vi "Network Streams Chat Window Launcher Client.vi"() -> ()   [LabVIEW 2020]
uses:
  Chat Window/Chat Window.lvclass
  C:/Program Files/National Instruments/LabVIEW 2026/vi.lib/ActorFramework/Actor/Actor.lvclass
  Protocols/Network Stream Strategy/Network Stream/Network Stream.lvclass/Network Stream.ctl
  Protocols/Network Stream Strategy/Network Stream Initiator/Network Stream Initiator.lvclass/Network Stream Initiator.ctl
  Chat Window/Chat Window.lvclass/Chat Window.ctl
  Protocols/Network Stream Strategy/Network Stream Initiator/Network Stream Initiator.lvclass
  C:/Data/1_Projects/network-endpoint-actors/Source/Protocols/Network Stream Strategy/Network Stream/Network Stream.lvclass
  C:/Data/1_Projects/network-endpoint-actors/Source/Abstract Classes/Message Stream/Message Stream.lvclass
  <vilib>/ActorFramework/Actor/Actor.lvclass
panel:
  in  "Listener Name":string="Bob"
  in  "Address":string="127.0.0.1"
  in  "Initiator Name":string="Fred"
  out "error out":errorcluster
  # "This VI launches two instances of a chat window actor.  The two chat windows launch nested endpoints, which connect via a Network Stream mesage stream.\n\n1.  (Optional)  Specify the IP address for this machine, and the names of the two stream endpoints\n2.  Run this VI.\n3.  Stop the application by closing either chat window.\n\nAF_Debug_Trace is set to TRUE in this project, so you can follow the action with the Desktop Execution Trace Toolkit."
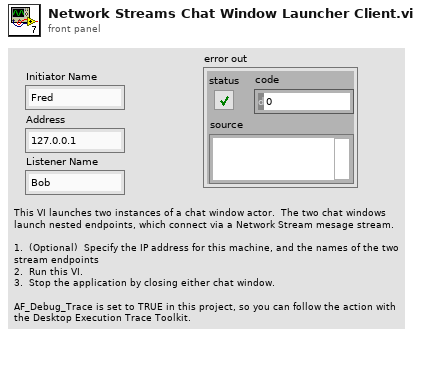
[diagram p1: front panel]
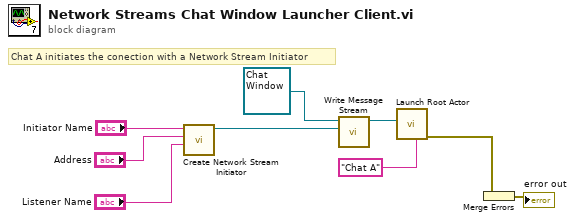
[diagram p0: block diagram]
diagram:
  # "Chat A initiates the conection with a Network Stream Initiator"
  n1 = call "Create Network Stream Initiator.vi"("Remote Name"="Listener Name", "Remote Address"="Address", "Name"="Initiator Name") -> ("Network Stream Initiator out"=w4:refnum<class "Network Stream Initiator.lvclass">)  [unwired: 8 in]
  n2 = call "Write Message Stream.vi"("Message Stream"=w4, "Chat Window in"=refnum<class "Chat Window.lvclass"> refnum) -> ("Chat Window out"=w8:refnum<class "Chat Window.lvclass">)  [unwired: 9 in]
  n3 = call <vilib>:"Launch Root Actor.vi"("Debug Alias"="Chat A", "Actor"=w8) -> ("error out"=w6:errorcluster)  [unwired: 8 in, 1 out]
  n4 = Merge Errors(w6) -> (→"error out":errorcluster)
